vi "ActionVIOnDownload.vi"(5 "System Definition Dir":path, 7 "Details Ref":refnum<vi>, 8 "error in (no error)":errorcluster, 10 "SFTP session in":refnum<class "Session.lvclass">, 11 "Device Item Ref in":T1 format="%.0x") -> (0 "error out":errorcluster, 2 "SFTP session out":refnum<class "Session.lvclass">, 3 "Device Item Ref out":T1 format="%.0x")   [LabVIEW 2027, in "System Monitor System Explorer.lvlib"]
uses:
  System Monitor System Explorer.lvlib
  <vilib>/NI VeriStand/Custom Device API/Custom Device Item Ref.ctl
  <vilib>/net/SFTP/Session/Session.lvclass
  <vilib>/net/SFTP/Session/Session.lvclass/Session.ctl
  <vilib>/net/SFTP/Session/Read user_host.vi
  C:/Program Files/National Instruments/VeriStand 2027/NationalInstruments.VeriStand.SystemDefinitionAPI.dll
  Program Files/National Instruments/VeriStand 2027/NationalInstruments.VeriStand.SystemDefinitionAPI.dll
  C:/Program Files/National Instruments/VeriStand 2027/NationalInstruments.VeriStand.SystemStorage.dll
  Program Files/National Instruments/VeriStand 2027/NationalInstruments.VeriStand.SystemStorage.dll
  <vilib>/NI VeriStand/Custom Device Tools/Custom Device Utility Library/Custom Device Utility Library.lvlib
  C:/Program Files/National Instruments/VeriStand 2027/NationalInstruments.VeriStand.dll
  Program Files/National Instruments/VeriStand 2027/NationalInstruments.VeriStand.dll
  <vilib>/NI VeriStand/Custom Device API/Custom Device API.lvlib
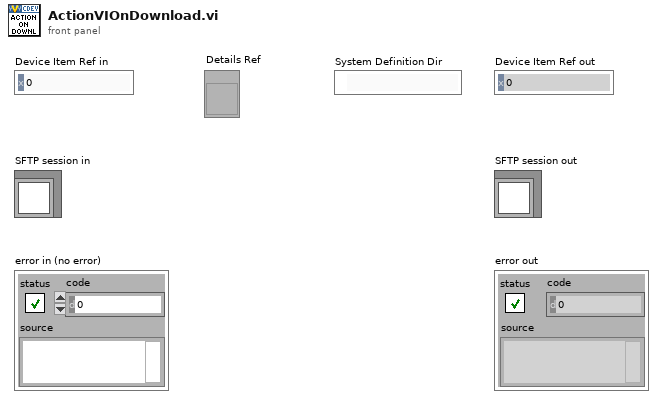
[diagram p1: front panel]
types:
  T1 = typedef "Custom Device API.lvlib/Custom Device Item Ref.ctl" = u64
  T2 = enum16{"open", "replace", "create", "open or create", "replace or create", "replace or create with confirmation"}
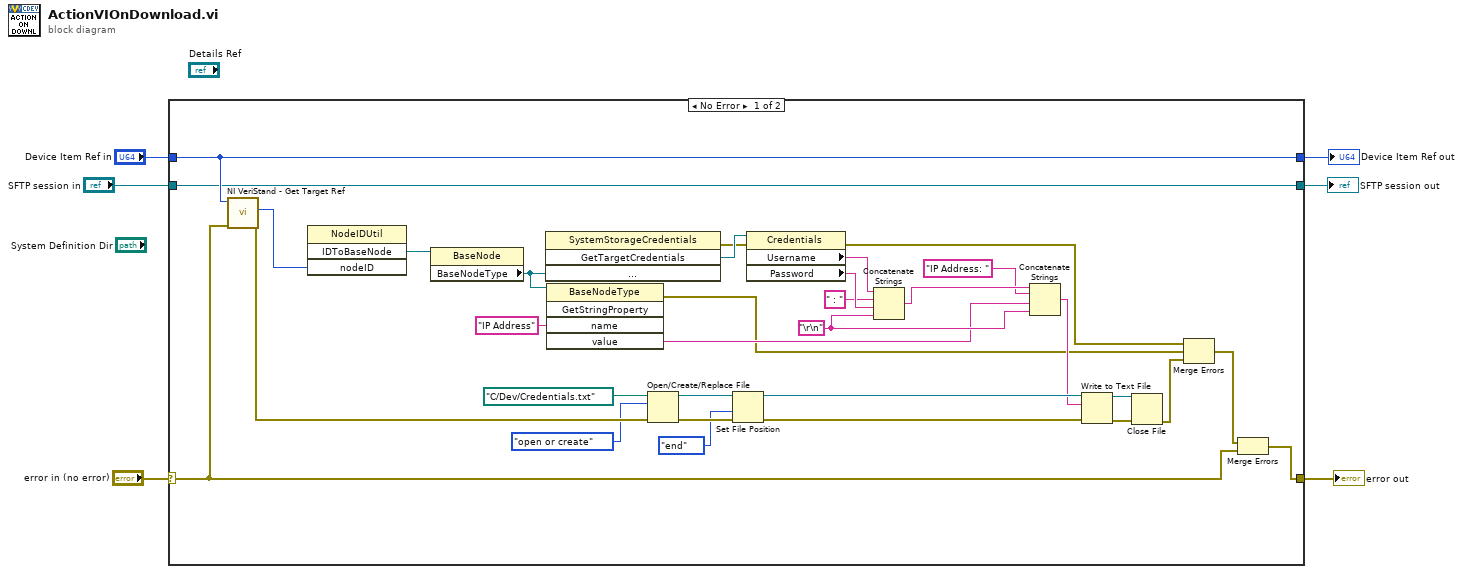
[diagram p0: block diagram]
diagram:
  n1 = case shown="No Error" "error in (no error)" {
    selector: "error in (no error)" -> [w20 w41]
    tunnel: [w19 w41] -> w5
    tunnel: "SFTP session in" -> [w18 w40]
    tunnel: [w18 w40] -> w1
    tunnel: "Device Item Ref in" -> [w38 w39]
    tunnel: [w38 w39] -> w3
    frame No Error {
      w12 = "\r\n"
      n2 = call <vilib>:"NI VeriStand - Get Target Ref.vi"("error in"=w20, "Item Ref in"=w38) -> ("error out"=w31:errorcluster, "Target Ref"=w15:T1)  [unwired: 6 in, 2 out]
      n3 = invoke class="NodeIDUtil" method="IDToBaseNode"("nodeID"=w15) -> ("IDToBaseNode"=w8:refnum<k39>)  [unwired: 3 in, 3 out]
      n4 = property class="BaseNode"(reference=w8) -> ("BaseNodeType"=w7:refnum<k39>)  [unwired: 1 in, 2 out]
      n5 = invoke class="SystemStorageCredentials" method="GetTargetCredentials"("targetNode"=w7) -> (error out=w36:errorcluster, "GetTargetCredentials"=w37:refnum<k39>)  [unwired: 3 in, 2 out]
      n6 = invoke class="BaseNodeType" method="GetStringProperty"(reference=w7, "name"="IP Address") -> (error out=w9:errorcluster, "value"=w11:string)  [unwired: 3 in, 3 out]
      n7 = Open/Create/Replace File(file path (use dialog)=path "C:/Dev/Credentials.txt", error in=w31, operation (0:open)=T2."open or create") -> (refnum out=w30:refnum<file>, error out=w32:errorcluster)  [unwired: 3 in, 1 out]
      n8 = Set File Position(refnum=w30, from (0:start)=enum16{"start", "end", "current"}."end", error in=w32) -> (refnum out=w35:refnum<file>, error out=w29:errorcluster)  [unwired: 1 in]
      n9 = property class="Credentials"(reference=w37, error in=w36) -> (error out=w10:errorcluster, "Username"=w27:string, "Password"=w26:string)  [unwired: 1 out]
      n10 = Concatenate Strings(w27, " : " ("string"), w26, w12) -> (w16:string)
      n11 = Concatenate Strings(w16, "IP Address: " ("string"), w11, w12) -> (w17:string)
      n12 = Write to Text File(file (use dialog)=w35, text=w17, error in=w29) -> (refnum out=w34:refnum<file>, error out=w28:errorcluster)  [unwired: 1 in, 1 out]
      n13 = Close File(refnum=w34, error in=w28) -> (error out=w22:errorcluster)  [unwired: 1 out]
      n14 = Merge Errors(w10, w9, w22) -> (w21:errorcluster)
      n15 = Merge Errors(w21, w20) -> (w19:errorcluster)
    }
    frame Error {
    }
  }
  "error out" <- w5
  "Device Item Ref out" <- w3
  "SFTP session out" <- w1
